vi "Gen_start.vi"(4 "Offset":dbl=0.001 min=0.0 max=3.3, 5 "Duty":u8 max=100, 6 "Amplitud":dbl=0.001 min=0.0 max=3.3, 7 "Frecuencia (Hz)":dbl=0.001 min=0.001 max=2000.0, 8 "error in (no error)":errorcluster, 9 "Tipo de Onda":u16(ring) items=["Senoidal", "Triangular", "Cuadrada", "Sierra"], 10 "Canal":u8, 11 "VISA resource name":refnum<visa-resource-name>) -> (0 "error out":errorcluster, 2 "respuesta":string, 3 "VISA resource name out":refnum<visa-resource-name>)   [LabVIEW 2026]
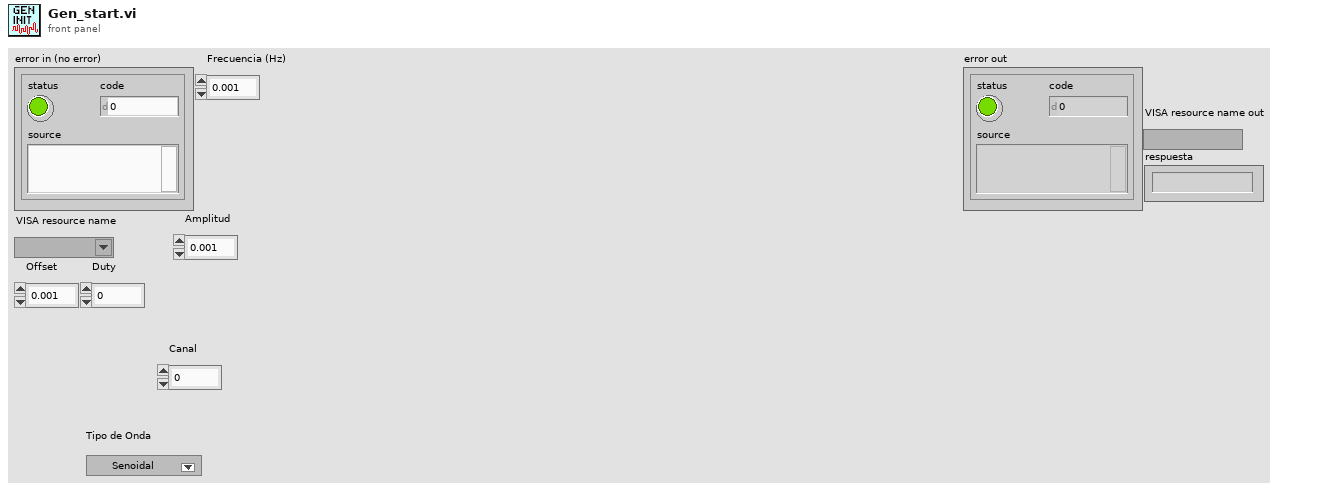
[diagram p1: front panel]
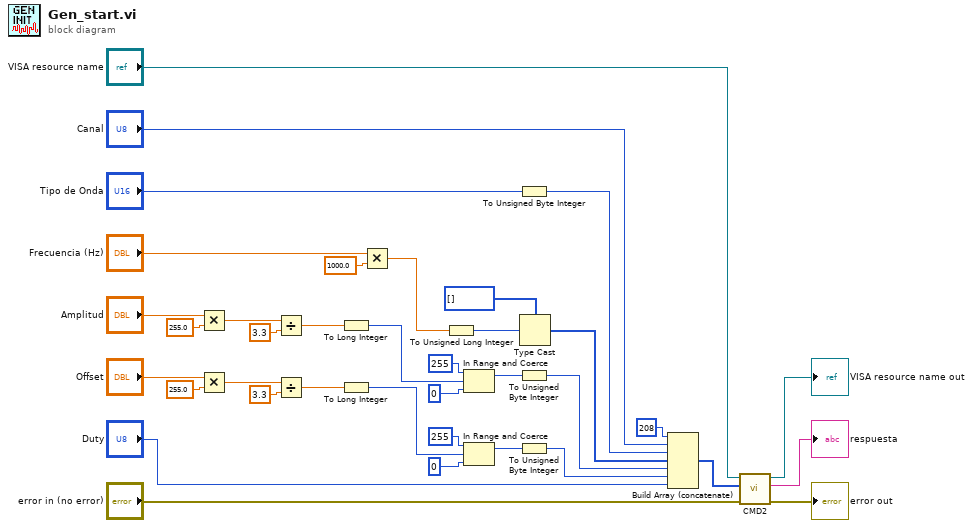
[diagram p0: block diagram]
diagram:
  n1 = Multiply(x="Amplitud", y=255.0) -> (x*y=w19:dbl)
  n2 = Multiply(x="Offset", y=255.0) -> (x*y=w8:dbl)
  n3 = Divide(x=w19, y=3.3) -> (x/y=w14:dbl)
  n4 = Divide(x=w8, y=3.3) -> (x/y=w13:dbl)
  n5 = To Long Integer(number=w14) -> (32bit integer=w15:i32)
  n6 = To Long Integer(number=w13) -> (32bit integer=w12:i32)
  n7 = Multiply(x="Frecuencia (Hz)", y=1000.0) -> (x*y=w25:dbl)
  n8 = To Unsigned Long Integer(number=w25) -> (unsigned 32bit integer=w24:u32)
  n9 = In Range and Coerce(upper limit=255, x=w15, lower limit=0) -> (coerced(x)=w5:i32)  [unwired: 1 out]
  n10 = In Range and Coerce(upper limit=255, x=w12, lower limit=0) -> (coerced(x)=w4:i32)  [unwired: 1 out]
  n11 = To Unsigned Byte Integer(number="Tipo de Onda") -> (unsigned 8bit integer=w28:u8)
  n12 = To Unsigned Byte Integer(number=w5) -> (unsigned 8bit integer=w3:u8)
  n13 = To Unsigned Byte Integer(number=w4) -> (unsigned 8bit integer=w2:u8)
  n14 = Type Cast(type=u8[] [], x=w24) -> (*(type *) &x=w22:u8[])
  n15 = Build Array (concatenate)(u8 208, "Canal", w28, w22, w3, w2, "Duty") -> (w31:u8[])
  n16 = call "CMD2.vi"("error in (no error)"="error in (no error)", "Comando"=w31, "VISA resource name"="VISA resource name") -> ("error out"=→"error out":errorcluster, "respuesta"=→"respuesta":string, "VISA resource name out"=→"VISA resource name out":refnum<visa-resource-name>)  [unwired: 6 in]
